vi "trim_to_bin.vi"(8 "number":u32, 11 "constant":u32) -> (0 "deleted portion":bool[](array[boolean]), 3 "new array":bool[](array[boolean]))   [LabVIEW 2025]
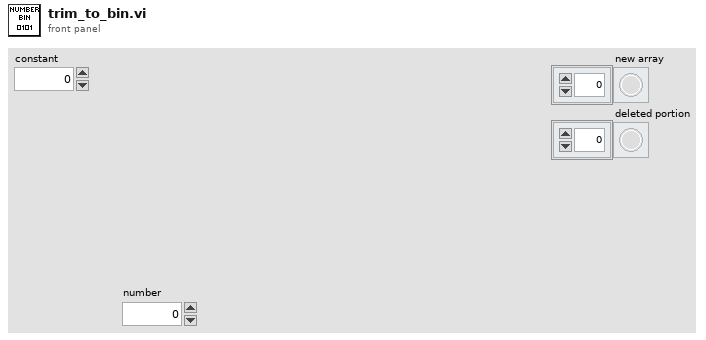
[diagram p1: front panel]
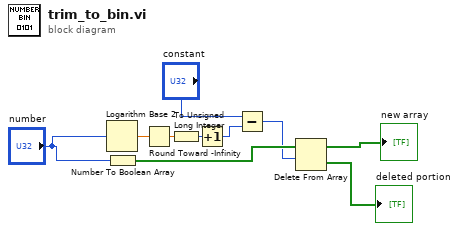
[diagram p0: block diagram]
diagram:
  n1 = Logarithm Base 2(1:"number") -> (0:w10:dbl)
  n2 = Number To Boolean Array(number="number") -> (Boolean array=w9:bool[])
  n3 = Round Toward -Infinity(1:w10) -> (0:w4:dbl)
  n4 = To Unsigned Long Integer(number=w4) -> (unsigned 32bit integer=w3:u32)
  n5 = Increment(x=w3) -> (x+1=w7:u32)
  n6 = Subtract(x="constant", y=w7) -> (x-y=w8:u32)
  n7 = Delete From Array(array=w9, length=w8) -> (deleted portion=→"deleted portion":bool[], array with subset deleted=→"new array":bool[])  [unwired: 1 in]
